vi "Signal_B_Table.vi"(8 "CP A Tag AZ":string[](array[string]), 11 "CP Profile Table for Bseq":string[][](table)) -> (3 "ACP Table":string[][](table) caption="LCP Table")   [LabVIEW 2018]
panel:
  out "Signal Intensity [pA]":string[](array[string])
  out "subarray":string[](array[string])
  out "Relative Assigned Level":string[](array[string])
  out "CP Length [ms]":string[](array[string])
  out "Assigned Base":string[](array[string])
  out "Direction":string[](array[string])
  out "Relative Averaged Data":string[](array[string])
  out "S#":string[](array[string])
  out "MS_IDX":string[](array[string])
  out "L#":string[](array[string])
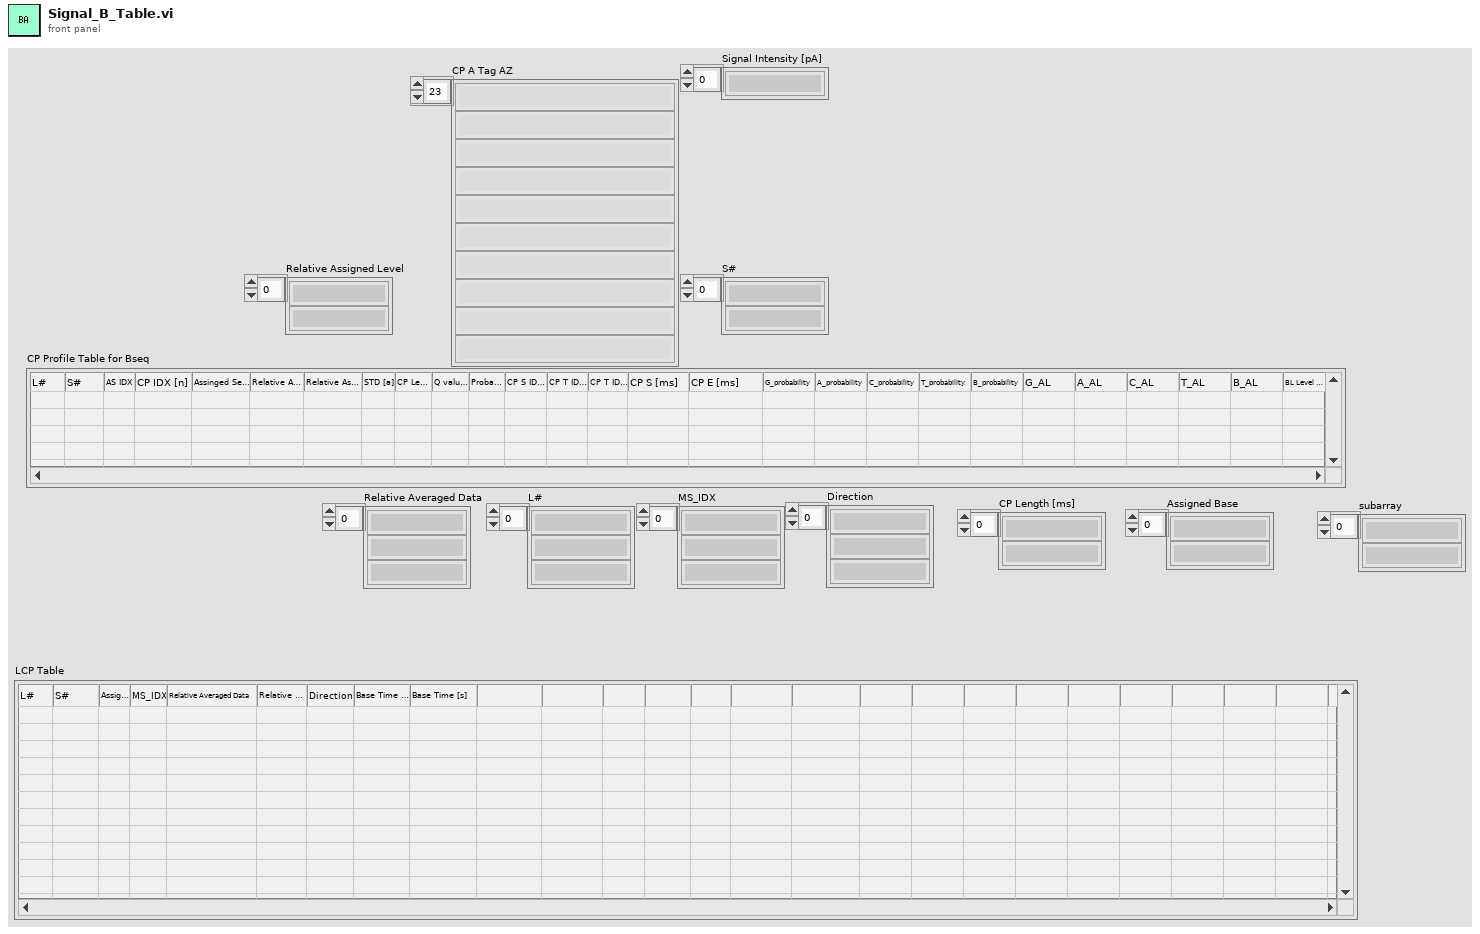
[diagram p1: front panel]
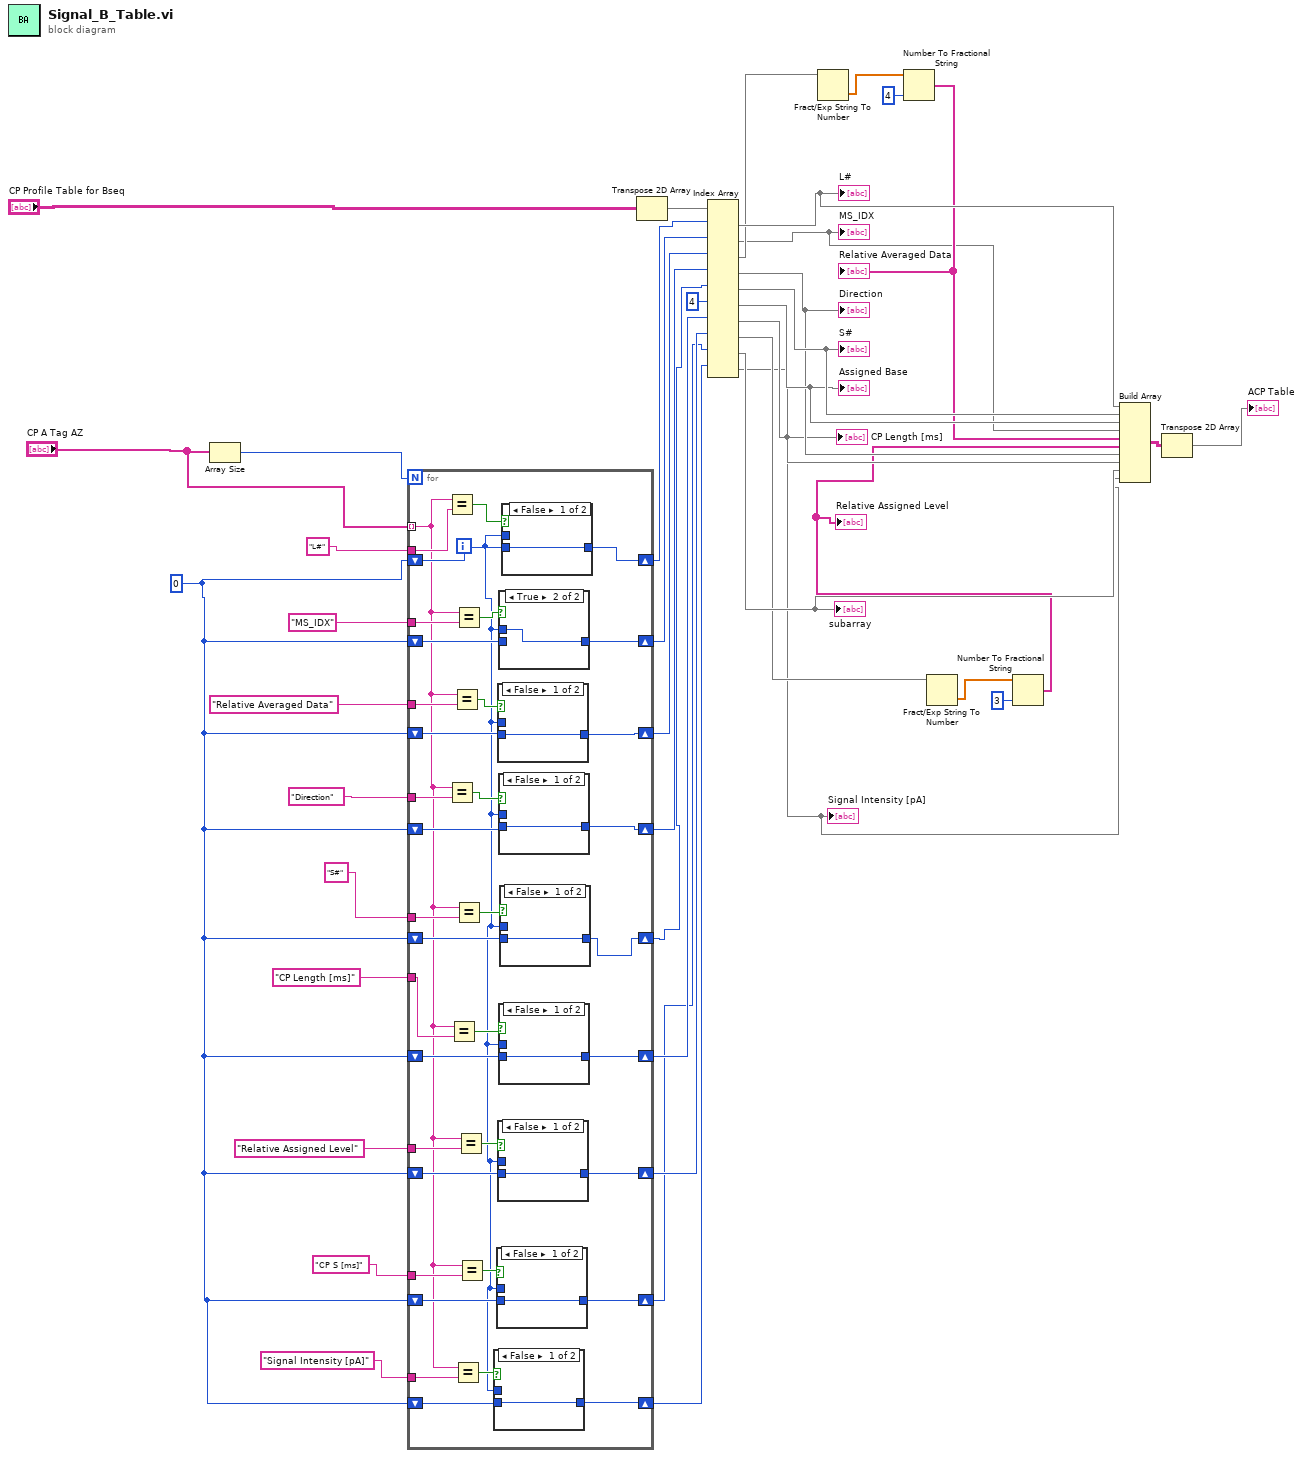
[diagram p0: block diagram]
diagram:
  w5 = 0 ("index (row)")
  n1 = Array Size(array="CP A Tag AZ") -> (size(s)=w41:i32)
  n2 = for {
    N: w41 -> [_]
    tunnel: "CP A Tag AZ" -> [w48] mode=indexing
    tunnel: "L#" ("y") -> [w80]
    shift-right: [w78] -> w35
    shift-left: w5 -> [w79]
    shift-right: [w75] -> w34
    shift-left: w5 -> [w76]
    shift-right: [w73] -> w33
    shift-left: w5 -> [w74]
    shift-right: [w71] -> w32
    shift-left: w5 -> [w72]
    tunnel: "MS_IDX" ("y") -> [w69]
    tunnel: "Relative Averaged Data" ("y") -> [w68]
    tunnel: "Direction" ("y") -> [w67]
    tunnel: "S#" ("y") -> [w63]
    shift-right: [w62] -> w30
    shift-left: w5 -> [w61]
    shift-right: [w59] -> w27
    shift-left: w5 -> [w60]
    tunnel: "CP Length [ms]" ("y") -> [w58]
    tunnel: "Relative Assigned Level" ("y") -> [w55]
    shift-right: [w53] -> w25
    shift-left: w5 -> [w54]
    shift-right: [w51] -> w23
    shift-left: w5 -> [w50]
    tunnel: "CP S [ms]" ("y") -> [w49]
    shift-right: [w44] -> w3
    shift-left: w5 -> [w45]
    tunnel: "Signal Intensity [pA]" ("y") -> [w43]
    i -> [w46]
    n3 = Equal?(x=w48, y=w80) -> (x = y?=w77:bool)
    n4 = Equal?(x=w48, y=w67) -> (x = y?=w65:bool)
    n5 = Equal?(x=w48, y=w58) -> (x = y?=w57:bool)
    n6 = Equal?(x=w48, y=w68) -> (x = y?=w66:bool)
    n7 = Equal?(x=w48, y=w43) -> (x = y?=w47:bool)
    n8 = Equal?(x=w48, y=w69) -> (x = y?=w70:bool)
    n9 = Equal?(x=w48, y=w63) -> (x = y?=w64:bool)
    n10 = Equal?(x=w48, y=w55) -> (x = y?=w56:bool)
    n11 = Equal?(x=w48, y=w49) -> (x = y?=w52:bool)
    n12 = case shown="False" w47 {
      tunnel: w46 -> [_ w82]
      tunnel: [w81 w82] -> w44
      tunnel: w45 -> [w81 _]
      frame False {
      }
      frame True {
      }
    }
    n13 = case shown="False" w52 {
      tunnel: w46 -> [_ w84]
      tunnel: [w83 w84] -> w51
      tunnel: w50 -> [w83 _]
      frame False {
      }
      frame True {
      }
    }
    n14 = case shown="False" w66 {
      tunnel: w46 -> [_ w94]
      tunnel: [w93 w94] -> w73
      tunnel: w74 -> [w93 _]
      frame False {
      }
      frame True {
      }
    }
    n15 = case shown="False" w56 {
      tunnel: w46 -> [_ w86]
      tunnel: [w85 w86] -> w53
      tunnel: w54 -> [w85 _]
      frame False {
      }
      frame True {
      }
    }
    n16 = case shown="True" w70 {
      tunnel: w46 -> [_ w96]
      tunnel: [w95 w96] -> w75
      tunnel: w76 -> [w95 _]
      frame False {
      }
      frame True {
      }
    }
    n17 = case shown="False" w65 {
      tunnel: w46 -> [_ w92]
      tunnel: [w91 w92] -> w71
      tunnel: w72 -> [w91 _]
      frame False {
      }
      frame True {
      }
    }
    n18 = case shown="False" w57 {
      tunnel: w46 -> [_ w88]
      tunnel: [w87 w88] -> w59
      tunnel: w60 -> [w87 _]
      frame False {
      }
      frame True {
      }
    }
    n19 = case shown="False" w64 {
      tunnel: w46 -> [_ w90]
      tunnel: [w89 w90] -> w62
      tunnel: w61 -> [w89 _]
      frame False {
      }
      frame True {
      }
    }
    n20 = case shown="False" w77 {
      tunnel: w46 -> [_ w98]
      tunnel: [w97 w98] -> w78
      tunnel: w79 -> [w97 _]
      frame False {
      }
      frame True {
      }
    }
  }
  n21 = Transpose 2D Array(2D array="CP Profile Table for Bseq") -> (transposed array=w42:string[][])
  n22 = Index Array(array=w42, index (row) #1=w35, index (row) #2=w34, index (row) #3=w33, index (row) #4=w32, index (row) #5=w30, index (row) #6=4 ("index (row)"), index (row) #7=w27, index (row) #8=w25, index (row) #9=w23, index (row) #10=w3) -> (element #1=w19:string[], element #2=w1:string[], element #3=w7:string[], element #4=w16:string[], element #5=w18:string[], element #6=w17:string[], element #7=w15:string[], element #8=w11:string[], element #9=w14:string[], element #10=w2:string[])  [unwired: 10 in]
  "L#" <- w19
  "MS_IDX" <- w1
  "S#" <- w18
  "Direction" <- w16
  "Assigned Base" <- w17
  "CP Length [ms]" <- w15
  "subarray" <- w14
  "Signal Intensity [pA]" <- w2
  n23 = Fract/Exp String To Number(string=w7) -> (number=w8:dbl[])  [unwired: 3 in, 1 out]
  n24 = Number To Fractional String(number=w8, precision (6)=i16 4) -> (F-format string=w6:string[])  [unwired: 2 in]
  "Relative Averaged Data" <- w6
  n25 = Fract/Exp String To Number(string=w11) -> (number=w12:dbl[])  [unwired: 3 in, 1 out]
  n26 = Number To Fractional String(number=w12, precision (6)=i16 3) -> (F-format string=w10:string[])  [unwired: 2 in]
  "Relative Assigned Level" <- w10
  n27 = Build Array(w19, w18, w17, w1, w6, w10, w16, w15, w14, w2) -> (w21:string[][])
  n28 = Transpose 2D Array(2D array=w21) -> (transposed array=→"ACP Table":string[][])
